vi "ReadWrite.ProcessData.vi"(8 "error in (no error)":errorcluster, 10 "timeout ms":i32=100, 11 "ReadWrite in":refnum<class "ReadWrite.lvclass">) -> (0 "error out":errorcluster, 1 "Timeout?":bool, 2 "Values":dbl[](array[numeric]), 3 "ReadWrite out":refnum<class "ReadWrite.lvclass">, 5 "Detect?":bool[](array[boolean]))   [LabVIEW 2015, in "Data Access Engine.lvlib" / "ReadWrite.lvclass"]
uses:
  ReadWrite.lvclass
  ReadWrite.lvclass/ReadWrite.ctl
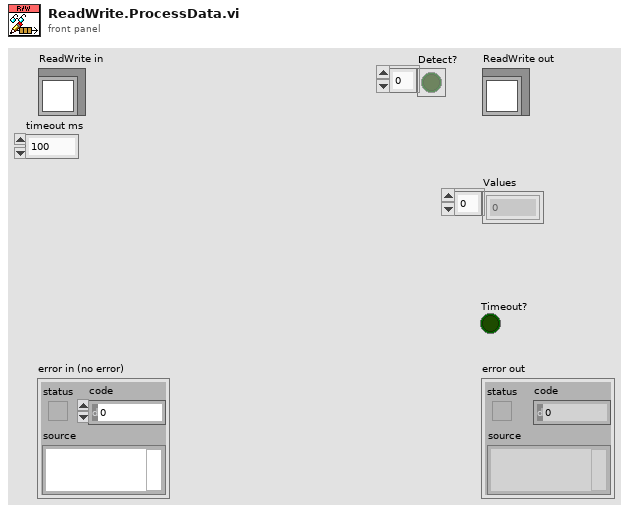
[diagram p1: front panel]
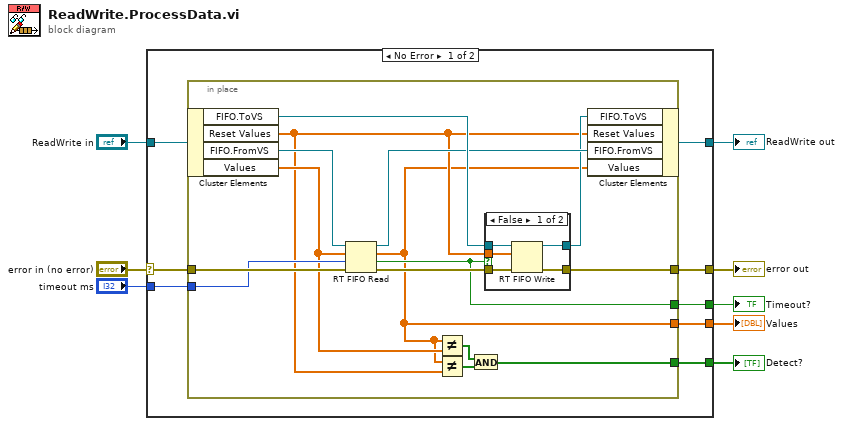
[diagram p0: block diagram]
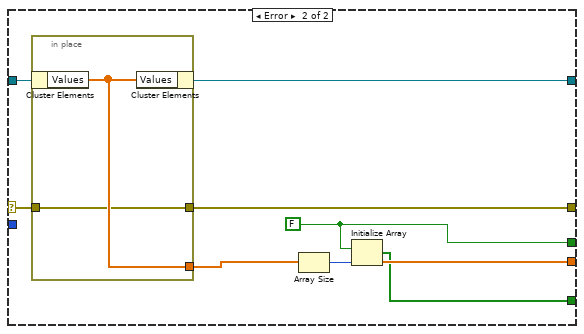
[diagram p3: hidden frame]
diagram:
  n1 = case shown="No Error" "error in (no error)" {
    selector: "error in (no error)" -> [w16 w43]
    tunnel: [w15 w44] -> w7
    tunnel: [w12 w45] -> w5
    tunnel: "ReadWrite in" -> [w13 w46]
    tunnel: [w14 w41] -> w4
    tunnel: "timeout ms" -> [w11 _]
    tunnel: [w10 w39] -> w2
    tunnel: [w9 w40] -> w1
    frame No Error {
      n2 = in-place {
        in-place-border: w16 -> [w30]
        in-place-border: [w25] -> w15
        in-place-border: [w19] -> w14
        in-place-border: w11 -> [w24]
        in-place-border: [w23] -> w10
        in-place-border: [w20] -> w9
        n3 = in-place-cluster #1(w13) -> ("FIFO.ToVS"=w28:refnum<k33>, "Reset Values"=w21:dbl[], "FIFO.FromVS"=w31:refnum<k33>, "Values"=w22:dbl[])
        n4 = RT FIFO Read(0:w31, 1:w22, 2:w24, 3:w30) -> (8:w27:refnum<k33>, 9:w19:dbl[], 10:w23:bool, 11:w29:errorcluster)  [unwired: 1 out]
        n5 = Not Equal?(x=w19, y=w22) -> (x != y?=w17:bool[])
        n6 = Not Equal?(x=w19, y=w21) -> (x != y?=w18:bool[])
        n7 = And(x=w17, y=w18) -> (x .and. y?=w20:bool[])
        n8 = case shown="False" w23 {
          tunnel: w29 -> [w36 w37]
          tunnel: w21 -> [w35 _]
          tunnel: w28 -> [w34 w38]
          tunnel: [w33 w38] -> w26
          tunnel: [w32 w37] -> w25
          frame False {
            n9 = RT FIFO Write(0:w34, 1:w35, 3:w36) -> (8:w33:refnum<k33>, 11:w32:errorcluster)  [unwired: 2 in, 2 out]
          }
          frame True {
          }
        }
        n10 = in-place-cluster #1("FIFO.ToVS"=w26, "Reset Values"=w21, "FIFO.FromVS"=w27, "Values"=w19) -> (w12:refnum<class "ReadWrite.lvclass">)
      }
    }
    frame Error {
      w39 = FALSE ("empty?")
      n11 = in-place {
        in-place-border: [w48] -> w41
        in-place-border: [w47] -> w44
        in-place-border: w43 -> [w47]
        n12 = in-place-cluster #2(w46) -> ("Values"=w48:dbl[])
        n13 = in-place-cluster #2("Values"=w48) -> (w45:refnum<class "ReadWrite.lvclass">)
      }
      n14 = Array Size(array=w41) -> (size(s)=w42:i32)
      n15 = Initialize Array(w39, w42) -> (w40:bool[])
    }
  }
  "error out" <- w7
  "ReadWrite out" <- w5
  "Values" <- w4
  "Timeout?" <- w2
  "Detect?" <- w1
